vi "StartCSMs.vi"(8 "error in":errorcluster, 11 "Array":T1(array[cluster])=[{"name"="Normal", "num"=1, "prototype"=[]}, {"name"=".SysLevel", "num"=1, "prototype"=[]}, {"name"="Normal.SubModule", "num"=1, "prototype"=[]}, {"name"="Normal2", "num"=1, "prototype"=[]}, {"name"=".SysLevel2", "num"=1, "prototype"=[]}, {"name"="Normal.SubModule2", "num"=1, "prototype"=[]}, {"name"="worker", "num"=3, "prototype"=[]}, {"name"="worker2", "num"=3, "prototype"=[]}, {"name"="Chain", "num"=1, "prototype"=[]}, {"name"="Chain", "num"=1, "prototype"=[]}, {"name"="Chain", "num"=1, "prototype"=[]}, {"name"="lvlibp", "num"=1, "prototype"=[]}, {"name"="lvlibp2", "num"=1, "prototype"=[]}]) -> (0 "error out":errorcluster, 2 "CSMs":string[](array[string]))   [LabVIEW 2017]
uses:
  src/user.lib/_NEVSTOP/Communicable State Machine(CSM)/Communicable State Machine.lvlib
  src/user.lib/_NEVSTOP/Communicable State Machine(CSM)/_Shared/CSM Shared.lvlib
panel:
  out "Waited (ms)":u32
  out "CSMs Left":string[](array[string])
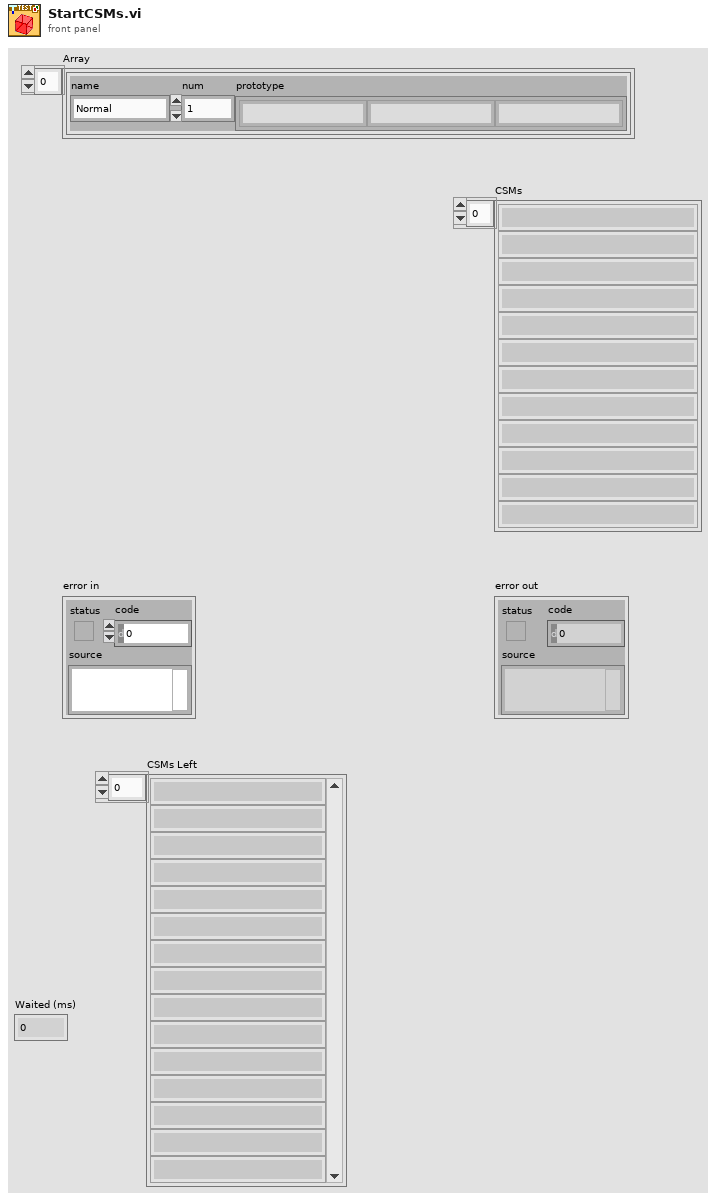
[diagram p1: front panel]
types:
  T1 = cluster{"name":string, "num":i32, "prototype":string[]}[]
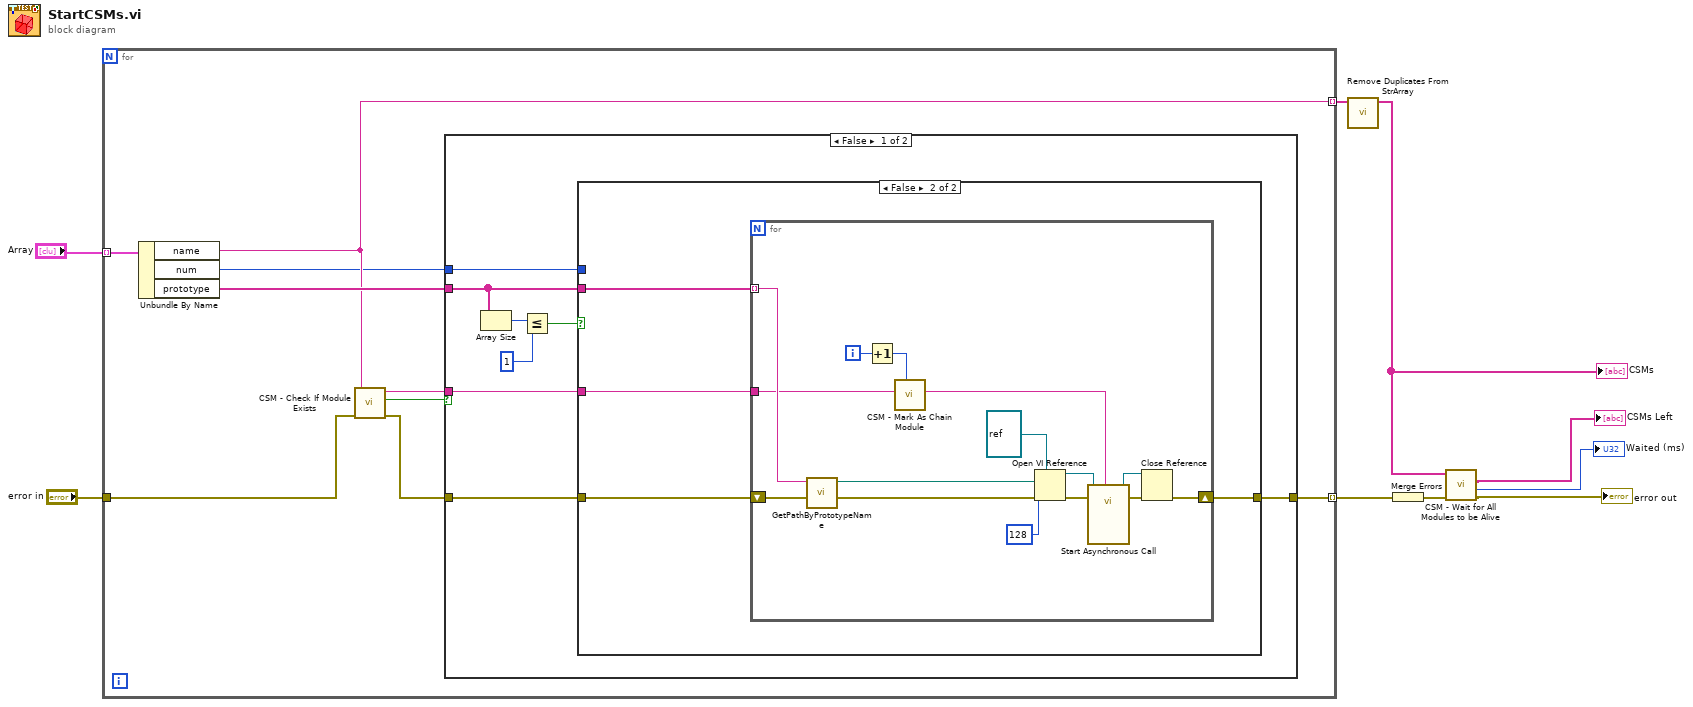
[diagram p0: block diagram]
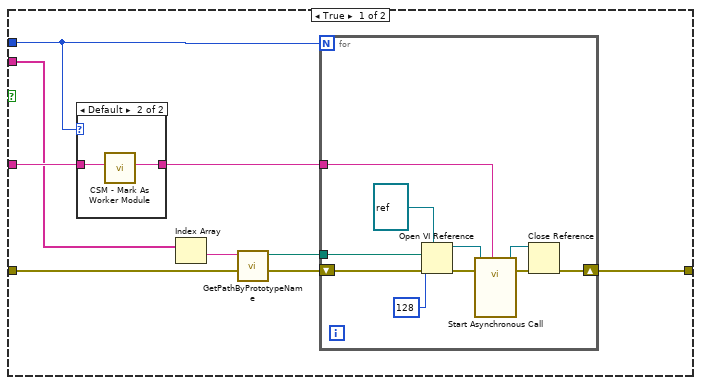
[diagram p2: hidden frame]
diagram:
  n1 = for {
    tunnel: [w18] -> w6 mode=indexing
    tunnel: "Array" -> [w14] mode=indexing
    tunnel: "error in" -> [w13]
    tunnel: [w11] -> w7 mode=indexing
    n2 = Unbundle By Name(w14) -> ("name"=w11:string, "num"=w10:i32, "prototype"=w12:string[])
    n3 = call "CSM - Check If Module Exists.vi"("Error In"=w13, "CSM Name"=w11) -> ("error out"=w17:errorcluster, "Exist?"=w15:bool, "CSM Name (Dup)"=w16:string)  [unwired: 7 in]
    n4 = case shown="False" w15 {
      tunnel: [w26 w66] -> w18
      tunnel: w17 -> [w25 w66]
      tunnel: w16 -> [w24 _]
      tunnel: w12 -> [w21 _]
      tunnel: w10 -> [w19 _]
      frame False {
        n5 = Array Size(array=w21) -> (size(s)=w23:i32)
        n6 = Less Or Equal?(x=w23, y=1) -> (x <= y?=w20:bool)
        n7 = case shown="False" w20 {
          tunnel: [w34 w51] -> w26
          tunnel: w25 -> [w33 w50]
          tunnel: w24 -> [w31 w49]
          tunnel: w21 -> [w30 w48]
          tunnel: w19 -> [w28 _]
          frame True {
            n8 = case shown="Default" w28 {
              tunnel: w31 -> [w45 w47]
              tunnel: [w45 w46] -> w32
              frame 0, 1 {
              }
              frame Default {
                n9 = call "CSM - Mark As Worker Module.vi"("CSM Name"=w47) -> ("CSM Name (Marked As Worker)"=w46:string)  [unwired: 9 in]
              }
            }
            n10 = Index Array(array=w30) -> (element=w29:string)  [unwired: 1 in]
            n11 = call "GetPathByPrototypeName.vi"("prototype"=w29) -> ("path"=w27:path)  [unwired: 10 in]
            n12 = for {
              N: w28 -> [_]
              tunnel: w32 -> [w38]
              shift-right: [w39] -> w34
              shift-left: w33 -> [w36]
              tunnel: w27 -> [w35]
              n13 = Open VI Reference(type specifier VI Refnum (for type only)=refnum<vi> refnum, vi path=w35, options=128, error in (no error)=w36) -> (vi reference=w41:refnum<vi>, error out=w43:errorcluster)  [unwired: 2 in]
              n14 = call-by-ref "Start Asynchronous Call"(reference=w41, error in=w43, "Name (\"\" to Use UUID)"=w38) -> (reference out=w40:refnum<vi>, error out=w42:errorcluster)  [unwired: 11 in]
              n15 = Close Reference(reference=w40, error in (no error)=w42) -> (error out=w39:errorcluster)
            }
          }
          frame False {
            n16 = for {
              tunnel: w49 -> [w54]
              shift-right: [w65] -> w51
              shift-left: w50 -> [w64]
              tunnel: w48 -> [w62] mode=indexing
              i -> [w55]
              n17 = call "GetPathByPrototypeName.vi"("prototype"=w62) -> ("path"=w63:path)  [unwired: 10 in]
              n18 = Increment(x=w55) -> (x+1=w52:i32)
              n19 = call "CSM - Mark As Chain Module.vi"("Order"=w52, "CSM Name"=w54) -> ("CSM Name (Marked As Chain)"=w53:string)  [unwired: 8 in]
              n20 = Open VI Reference(type specifier VI Refnum (for type only)=refnum<vi> refnum, vi path=w63, options=128, error in (no error)=w64) -> (vi reference=w58:refnum<vi>, error out=w60:errorcluster)  [unwired: 2 in]
              n21 = call-by-ref "Start Asynchronous Call"(reference=w58, error in=w60, "Name (\"\" to Use UUID)"=w53) -> (reference out=w57:refnum<vi>, error out=w59:errorcluster)  [unwired: 11 in]
              n22 = Close Reference(reference=w57, error in (no error)=w59) -> (error out=w65:errorcluster)
            }
          }
        }
      }
      frame True {
      }
    }
  }
  n23 = call "Remove Duplicates From StrArray.vi"("StrArray In"=w7) -> ("StrArray"=w1:string[])  [unwired: 9 in, 1 out]
  "CSMs" <- w1
  n24 = Merge Errors(w6) -> (w5:errorcluster)
  n25 = call "CSM - Wait for All Modules to be Alive.vi"("Error In"=w5, "CSM Names"=w1) -> ("error out"=→"error out":errorcluster, "Waited (ms)"=→"Waited (ms)":u32, "CSMs Left"=→"CSMs Left":string[])  [unwired: 7 in]
